vi "FuncVI-WFGraph.vi"(5 "InstanceRef":T2, 9 "arg list":T1[](array[typedef])) -> (0 "error out":bool caption="Error", 3 "result":T1)   [LabVIEW 2021]
doc: "::: CalcExpress Toolkit :::\nCopyright (c) 2000-2026 Konstantin Shifershteyn. All rights reserved."
uses:
  cetypes.llb/CalcExpress Function Argument Info.ctl
  cetypes.llb/CalcExpress Instance RefNum.ctl
panel:
  in  "max arg num":i32=8
  in  "min arg num":i32
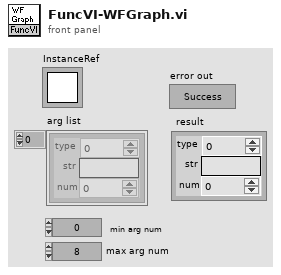
[diagram p1: front panel]
types:
  T1 = typedef "CalcExpress Function Argument Info.ctl" = cluster{"type":u32, "str":string, "num":dbl}
  T2 = typedef "CalcExpress Instance RefNum.ctl" = refnum<k1>
  T3 = cluster{"index":i32, "type":enum8{"String", "DBL Number", "identifier", "1D Array of DBL", "2D Array of DBL", "CDB Number", "1D Array of CDB", "2D Array of CDB", "Unknown data type"}, "default num":dbl, "default str":string}[]
  T4 = cluster{"data type":enum32{"String", "DBL Number", "identifier", "1D Array of DBL", "2D Array of DBL", "CDB Number", "1D Array of CDB", "2D Array of CDB", "1D Array of String", "2D Array of String", "Unknown data type"}, "str":string, "num":dbl}
  T5 = cluster{i32, "Sine Wave":dbl[], "str":dbl, "str":dbl, "str":string}
  T6 = cluster{"index":i32, "type":enum8{"String", "DBL Number", "identifier", "1D Array of DBL", "2D Array of DBL", "CDB Number", "1D Array of CDB", "2D Array of CDB", "Unknown data type"}, "default num":dbl, "default str":string}
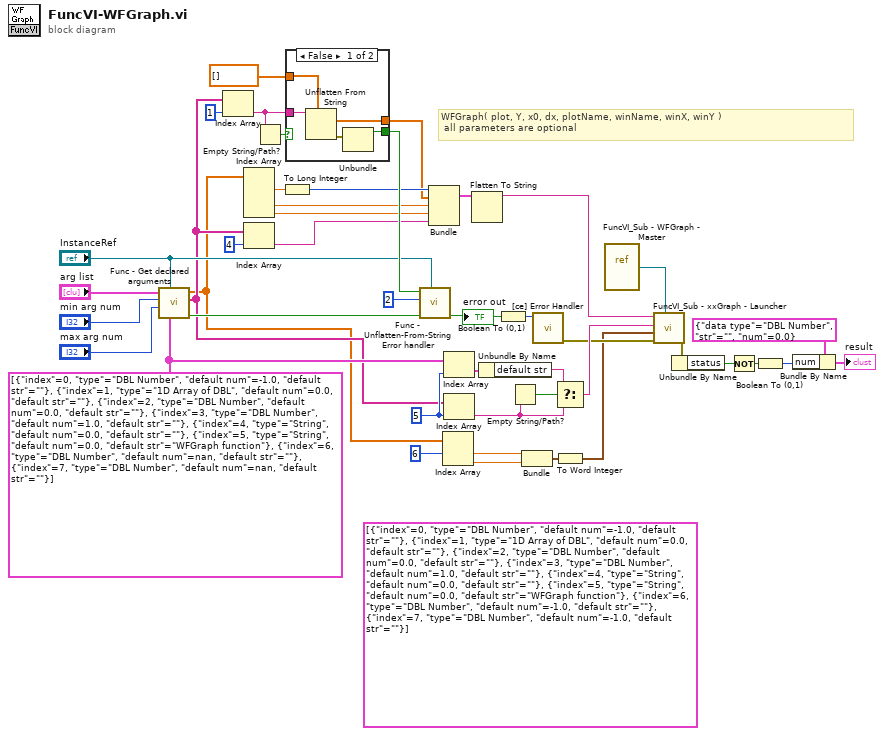
[diagram p0: block diagram]
diagram:
  (unwired) T3 [{"index"=0, "type"=enum."DBL Number", "default num"=-1.0, "default str"=""}, {"index"=1, "type"=enum."1D Array of DBL", "default num"=0.0, "default str"=""}, {"index"=2, "type"=enum."DBL Number", "default num"=0.0, "default str"=""}, {"index"=3, "type"=enum."DBL Number", "default num"=1.0, "default str"=""}, {"index"=4, "type"=enum."String", "default num"=0.0, "default str"=""}, {"index"=5, "type"=enum."String", "default num"=0.0, "default str"="WFGraph function"}, {"index"=6, "type"=enum."DBL Number", "default num"=-1.0, "default str"=""}, {"index"=7, "type"=enum."DBL Number", "default num"=-1.0, "default str"=""}] ("args descriptors")
  w24 = 5
  w6 = T3 [{"index"=0, "type"=enum."DBL Number", "default num"=-1.0, "default str"=""}, {"index"=1, "type"=enum."1D Array of DBL", "default num"=0.0, "default str"=""}, {"index"=2, "type"=enum."DBL Number", "default num"=0.0, "default str"=""}, {"index"=3, "type"=enum."DBL Number", "default num"=1.0, "default str"=""}, {"index"=4, "type"=enum."String", "default num"=0.0, "default str"=""}, {"index"=5, "type"=enum."String", "default num"=0.0, "default str"="WFGraph function"}, {"index"=6, "type"=enum."DBL Number", "default num"=nan, "default str"=""}, {"index"=7, "type"=enum."DBL Number", "default num"=nan, "default str"=""}] ("args descriptors")
  # "WFGraph( plot, Y, x0, dx, plotName, winName, winX, winY ) \n all parameters are optional"
  n1 = call "Func - Get declared arguments.vi"("arg descriptors"=w6, "InstanceRef"="InstanceRef", "max arg num"="max arg num", "min arg num"="min arg num", "arg list"="arg list") -> ("error out"=w37:bool, "str list"=w5:string[], "num list"=w4:dbl[])  [unwired: 3 in, 1 out]
  n2 = Index Array(array=w5, index=1) -> (element=w40:string)
  n3 = Index Array(array=w4) -> (element #1=w29:dbl, element #3=w28:dbl, element #4=w27:dbl)  [unwired: 4 in, 1 out]
  n4 = Index Array(array=w5, index=4) -> (element=w31:string)
  n5 = Empty String/Path?(string/path=w40) -> (empty?=w41:bool)
  n6 = To Long Integer(number=w29) -> (32bit integer=w32:i32)
  n7 = case shown="False" w41 {
    tunnel: [w49 _] -> w38
    tunnel: [w48 w50] -> w30
    tunnel: dbl[] [] ("Sine Wave") -> [w47 w50]
    tunnel: w40 -> [w46 _]
    frame False {
      n8 = Unflatten From String(type=w47, binary string=w46) -> (value=w48:dbl[], error out=w45:errorcluster)  [unwired: 3 in, 1 out]
      n9 = Unbundle(w45) -> ("status"=w49:bool)  [unwired: 2 out]
    }
    frame True {
    }
  }
  n10 = call "Func - Unflatten-From-String Error handler.vi"("InstanceRef"="InstanceRef", "error in"=w37, "argument number"=2, "Unflatten Error status"=w38) -> ("error out"=w2:bool)  [unwired: 5 in]
  "error out" <- w2
  n11 = Bundle(w32, "Sine Wave"=w30, "str"=w28, "str"=w27, "str"=w31) -> (w8:T5)  [unwired: 1 in]
  n12 = Index Array(array=w4, index #1=6) -> (element #1=w20:dbl, element #2=w21:dbl)  [unwired: 1 in]
  n13 = Index Array(array=w6, index=w24) -> (element=w10:T6)
  n14 = Index Array(array=w5, index=w24) -> (element=w25:string)
  n15 = Flatten To String(anything=w8) -> (data string=w9:string)  [unwired: 3 in, 2 out]
  n16 = Unbundle By Name(w10) -> ("default str"=w11:string)
  n17 = Boolean To (0,1)(Boolean=w2) -> (0, 1=w12:i16)
  n18 = Empty String/Path?(string/path=w25) -> (empty?=w23:bool)
  n19 = Bundle("str"=w20, "str"=w21) -> (w22:cluster{"str":dbl, "str":dbl})  [unwired: 1 in]
  n20 = call "[ce] Error Handler.vi"("error code"=w12) -> ("error out"=w13:errorcluster)  [unwired: 9 in, 1 out]
  n21 = Select(t=w11, s=w23, f=w25) -> (s? t:f=w26:string)
  n22 = To Word Integer(number=w22) -> (16bit integer=w7:cluster{"str":i16, "str":i16})
  n23 = vi-ref "FuncVI_Sub - WFGraph - Master.vi"() -> (w1:refnum<vi>)
  n24 = call "FuncVI_Sub - xxGraph - Launcher.vi"("Master VI Refnum"=w1, "error in"=w13, "left-top corner"=w7, "win name"=w26, "data"=w9) -> ("error out"=w18:errorcluster)  [unwired: 6 in]
  n25 = Unbundle By Name(w18) -> ("status"=w17:bool)
  n26 = Not(x=w17) -> (.not. x?=w14:bool)
  n27 = Boolean To (0,1)(Boolean=w14) -> (0, 1=w16:i16)
  n28 = Bundle By Name(cluster=T4 {"data type"=enum."DBL Number", "str"="", "num"=0.0} ("opd info"), "num"=w16) -> (→"result":T4)
